vi "reset SA Device.vi"(8 "error in (no error)":errorcluster, 11 "Keysight 9020A in":refnum<class "Keysight 9020A.lvclass">) -> (0 "error out":errorcluster, 3 "Keysight 9020A out":refnum<class "Keysight 9020A.lvclass">)   [LabVIEW 2023, in "Spectrum Analyzer.lvlib" / "Keysight 9020A.lvclass"]
uses:
  Keysight 9020A.lvclass
  Keysight 9020A.lvclass/Keysight 9020A.ctl
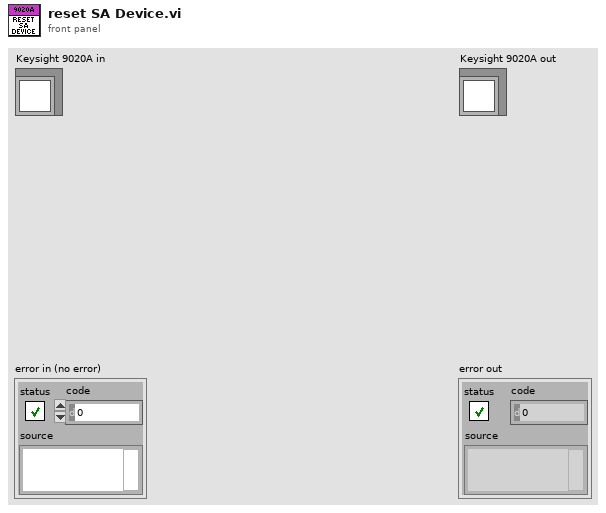
[diagram p1: front panel]
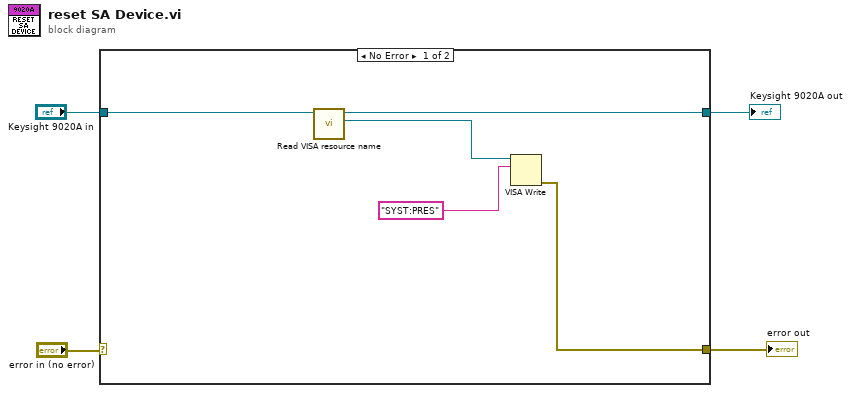
[diagram p0: block diagram]
diagram:
  n1 = case shown="No Error" "error in (no error)" {
    selector: "error in (no error)" -> [_ w10]
    tunnel: "Keysight 9020A in" -> [w6 w11]
    tunnel: [w9 w11] -> w3
    tunnel: [w7 w10] -> w1
    frame No Error {
      n2 = call "Read VISA resource name.vi"("Keysight 9020A in"=w6) -> ("VISA resource name"=w8:refnum<visa-resource-name>, "Keysight 9020A out"=w9:refnum<class "Keysight 9020A.lvclass">)  [unwired: 8 in, 1 out]
      n3 = VISA Write(VISA resource name=w8, write buffer="SYST:PRES") -> (error out=w7:errorcluster)  [unwired: 1 in, 2 out]
    }
    frame Error {
    }
  }
  "error out" <- w1
  "Keysight 9020A out" <- w3
